vi "New Client Handle.vi"(5 "http-client (default)":refnum<class "http-client.lvclass">, 8 "error in (no error)":errorcluster, 11 "REST Client in":refnum<class "REST Client.lvclass">) -> (0 "error out":errorcluster, 2 "http-client":refnum<class "http-client.lvclass">, 3 "REST Client out":refnum<class "REST Client.lvclass">)   [LabVIEW 2020, in "REST Client.lvlib" / "REST Client.lvclass"]
uses:
  REST Client.lvclass
  http-client/http-client.lvclass
  REST Client.lvclass/REST Client.ctl
  advanced-http-client/advanced-http-client.lvclass
  C:/Repositories/JKI/http-rest-client/source/classes/http-client/http-client.lvclass
  basic-http-client/basic-http-client.lvclass
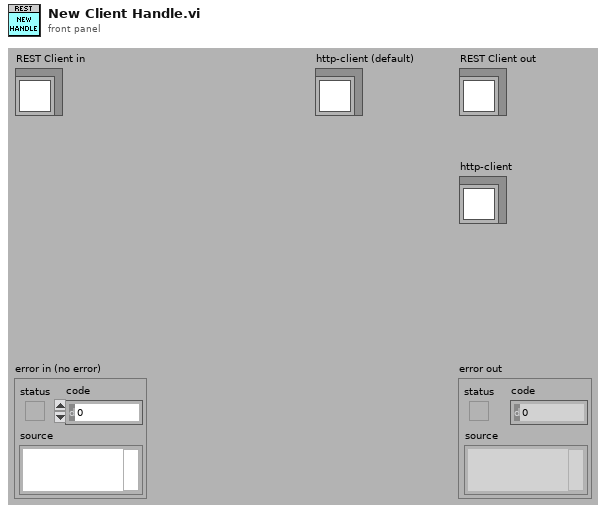
[diagram p1: front panel]
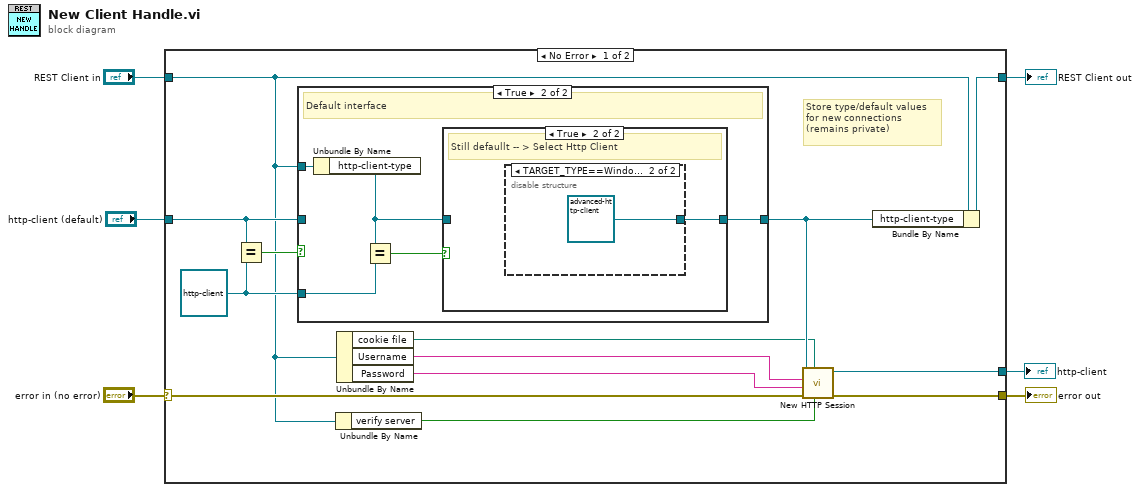
[diagram p0: block diagram]
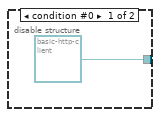
[diagram p4: hidden frame]
diagram:
  n1 = case shown="No Error" "error in (no error)" {
    selector: "error in (no error)" -> [w15 w31]
    tunnel: [w16 w31] -> w5
    tunnel: [w14 w30] -> w3
    tunnel: "REST Client in" -> [w8 w30]
    tunnel: [w17 _] -> w2
    tunnel: "http-client (default)" -> [w18 _]
    frame No Error {
      w13 = refnum<class "http-client.lvclass"> refnum ("http-client")
      # "Store type/default values \nfor new connections\n(remains private)"
      n2 = Equal?(x=w18, y=w13) -> (x = y?=w19:bool)
      n3 = case shown="True" w19 {
        tunnel: w18 -> [w20 _]
        tunnel: [w20 w25] -> w12
        tunnel: w8 -> [_ w24]
        tunnel: w13 -> [_ w23]
        frame False {
          # "Not default -- > Use the provided implementation"
        }
        frame True {
          # "Default interface"
          n4 = Unbundle By Name(w24) -> ("http-client-type"=w21:refnum<class "http-client.lvclass">)
          n5 = Equal?(x=w21, y=w23) -> (x = y?=w22:bool)
          n6 = case shown="True" w22 {
            tunnel: [w26 w27] -> w25
            tunnel: w21 -> [w26 _]
            frame False {
              # "Non-default -- > use it"
            }
            frame True {
              # "Still defaullt -- > Select Http Client"
              n7 = disable-structure shown="TARGET_TYPE==Windows" {
                disable-tunnel: [refnum<class "basic-http-client.lvclass"> refnum ("REST Client.lvlib:basic-http-client.lvclass") refnum<class "advanced-http-client.lvclass"> refnum ("REST Client.lvlib:advanced-http-client.lvclass")] -> w27
                frame condition #0 {
                }
                frame condition #1 (active) {
                }
              }
            }
          }
        }
      }
      n8 = Unbundle By Name(w8) -> ("verify server"=w7:bool)
      n9 = Unbundle By Name(w8) -> ("cookie file"=w11:path, "Username"=w10:string, "Password"=w9:string)
      n10 = call "New HTTP Session.vi"("verify server (true)"=w7, "cookie file"=w11, "error in (no error)"=w15, "password"=w9, "username"=w10, "http-client in"=w12) -> ("error out"=w16:errorcluster, "http-client out"=w17:refnum<class "http-client.lvclass">)  [unwired: 4 in]
      n11 = Bundle By Name(cluster=w8, "http-client-type"=w12) -> (w14:refnum<class "REST Client.lvclass">)
    }
    frame Error {
    }
  }
  "error out" <- w5
  "REST Client out" <- w3
  "http-client" <- w2
